vi "I2C Read.vi"(8 "error in (no error)":errorcluster, 10 "Size":i32=1, 11 "I2C Device":T1) -> (0 "error out":errorcluster, 2 "Values":u8[](array[numeric]), 3 "I2C Device out":T1)   [LabVIEW 2020, in "wiringPi.lvlib"]
doc: "<b>_______________________________________________________________</b>\n** Author: Juan José Villacorta\n** LabVIEW wrapper for C library <b> wiringPi </b>,\n** https://github.com/WiringPi/WiringPi\n<b>_______________________________________________________________</b>\n/*\n * Read data from the I2C device\n**********************************************************************************\n*/"
uses:
  wiringPi.lvlib
  Type Defs/I2C Device.ctl
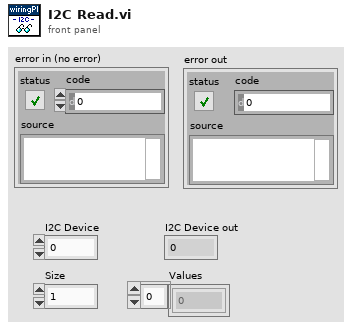
[diagram p1: front panel]
types:
  T1 = typedef "wiringPi.lvlib/I2C Device.ctl" = i32
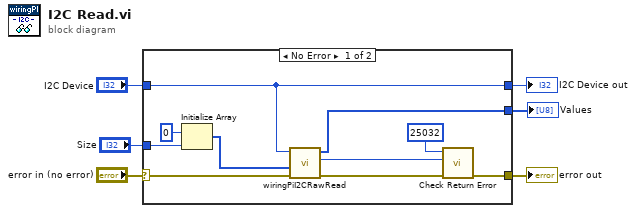
[diagram p0: block diagram]
diagram:
  n1 = case shown="No Error" "error in (no error)" {
    selector: "error in (no error)" -> [w15 w18]
    tunnel: [w16 w18] -> w5
    tunnel: "I2C Device" -> [w13 w17]
    tunnel: [w13 w17] -> w4
    tunnel: "Size" -> [w10 _]
    tunnel: [w7 _] -> w1
    frame No Error {
      n2 = Initialize Array(u8 0 ("element"), w10) -> (w9:u8[])
      n3 = call "wiringPiI2CRawRead.vi"("error in (no error)"=w15, "values"=w9, "devID"=w13) -> ("error out"=w14:errorcluster, "return"=w12:i32, "values readed"=w7:u8[])  [unwired: 6 in]
      n4 = call "Check Return Error.vi"("error in (no error)"=w14, "Return code"=w12, "Error number"=25032) -> ("error out"=w16:errorcluster)  [unwired: 8 in]
    }
    frame Error {
    }
  }
  "error out" <- w5
  "I2C Device out" <- w4
  "Values" <- w1
